vi "measure BT OCW Measurement.vi"(8 "error in (no error)":errorcluster, 11 "SA Measurement in":refnum<class "SA Measurement.lvclass">) -> (0 "error out":errorcluster, 3 "SA Measurement out":refnum<class "SA Measurement.lvclass">)   [LabVIEW 2023, in "Spectrum Analyzer.lvlib" / "SA Measurement.lvclass"]
uses:
  SA Measurement.lvclass
  SA Measurement.lvclass/SA Measurement.ctl
  TYPE DEFINITION/Keysight 9020A/TYPE Measurement Preset.ctl
  Spectrum Analyzer.lvlib
  TYPE DEFINITION/TYPE RBW and VBW Select.ctl
  Interface_Spectrum/Interface_Spectrum.lvclass
  TYPE DEFINITION/TYPE Marker Peak Search Type.ctl
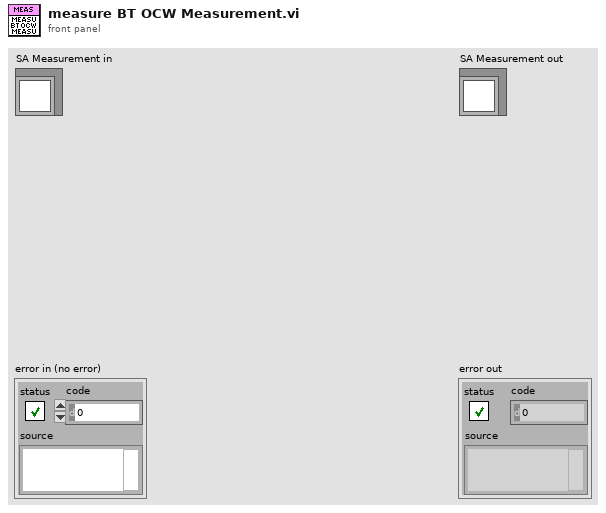
[diagram p1: front panel]
types:
  T1 = typedef "Spectrum Analyzer.lvlib/TYPE Marker Peak Search Type.ctl" = enum16{"Max", "Next Peak", "Max - Auto"}
  T2 = typedef "Spectrum Analyzer.lvlib/TYPE RBW and VBW Select.ctl" = enum16{"Res BW", "Video BW"}
  T3 = typedef "Spectrum Analyzer.lvlib/TYPE Measurement Preset.ctl" = enum16{"Sweep SA Mode", "Channel Power", "Occupied BW", "ACP", "Spurious Emission", "Spurious Emission Mask", "Burst Power (Transmit Power)"}
  T4 = typedef "Spectrum Analyzer.lvlib/TYPE Y-axis Unit.ctl" = enum16{"dBm", "dBmV", "dBuV", "dBpW", "Volt", "Ampere", "Watt"}
  T5 = typedef "Spectrum Analyzer.lvlib/TYPE Reference Level and Atten Param.ctl" = cluster{"Reference Level":dbl, "Atten":i32, "Atten Auto?":bool, "Reference Level Offset":dbl}
  T6 = typedef "Spectrum Analyzer.lvlib/TYPE Display Trace Mode Select.ctl" = enum16{"Clear Write", "Max Hold", "Min Hold", "Average", "View"}
  T7 = typedef "Spectrum Analyzer.lvlib/TYPE Detect Mode Select.ctl" = enum16{"Det Auto (Normal)", "Auto Peak", "Positive Peak", "Negative Peak", "Sample", "RMS", "Average", "Quasipeak", "CISPR Average", "RMS Average"}
  T8 = cluster{"Trace Mode":T6, "Detector Type":T7, "Detect Auto?":bool}[]
  T9 = typedef "Spectrum Analyzer.lvlib/TYPE Marker Value.ctl" = cluster{"X-axis":dbl, "Y-axis":dbl}
  T10 = typedef "Spectrum Analyzer.lvlib/TYPE OBW Measurement.ctl" = cluster{"Occupied BW (Hz)":dbl, "Total Power or OBW Power - dBm":dbl, "Transmit Frequency Error (Hz)":dbl, "x DB Bandwidth (Hz)":dbl, "Lower OBW Frequency (Hz)":dbl, "Upper OBW Frequency (Hz)":dbl}
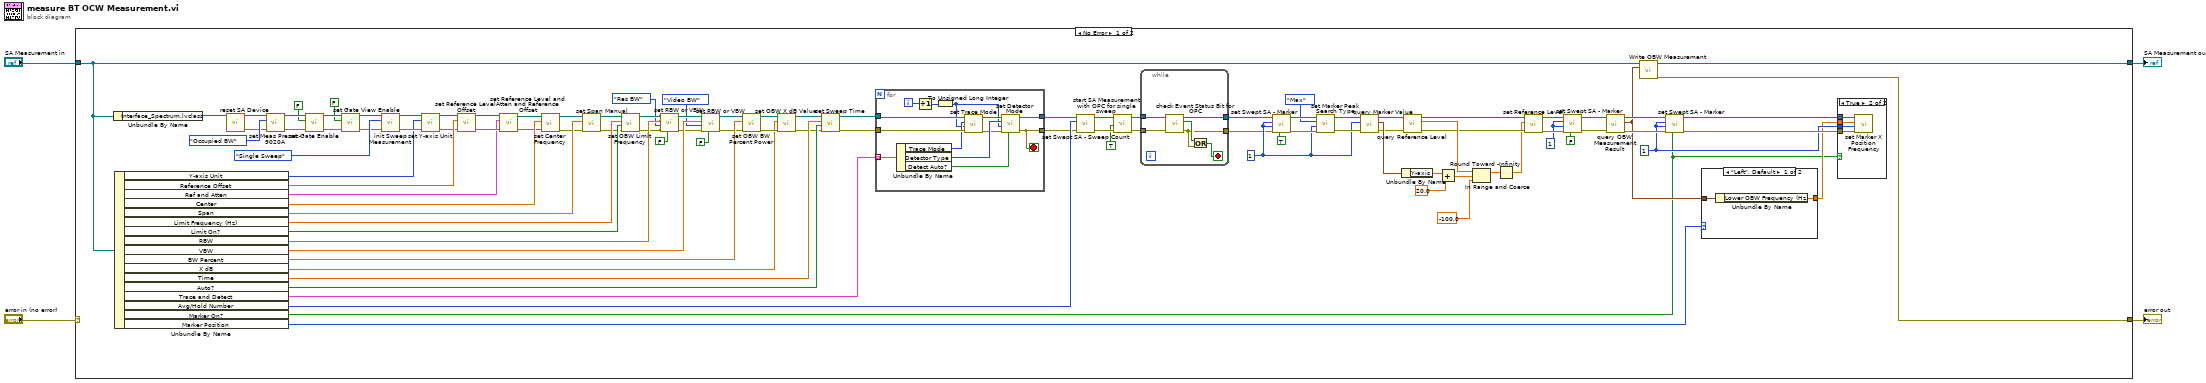
[diagram p0: block diagram]
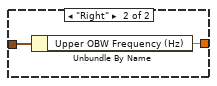
[diagram p3: hidden frame]
diagram:
  n1 = case shown="No Error" "error in (no error)" {
    selector: "error in (no error)" -> [_ w135]
    tunnel: [w58 w135] -> w3
    tunnel: [w59 w134] -> w1
    tunnel: "SA Measurement in" -> [w60 w134]
    frame No Error {
      w25 = 1 ("Index")
      w41 = 1 ("Index")
      w51 = 1 ("Index")
      n2 = Unbundle By Name(w60) -> ("Interface_Spectrum.lvclass"=w92:refnum<class "Interface_Spectrum.lvclass">)
      n3 = Unbundle By Name(w60) -> ("Y-axis Unit"=w100:T4, "Reference Offset"=w104:dbl, "Ref and Atten"=w8:T5, "Center"=w103:dbl, "Span"=w82:dbl, "Limit Frequency (Hz)"=w89:dbl, "Limit On?"=w88:bool, "RBW"=w77:dbl, "VBW"=w71:dbl, "BW Percent"=w87:dbl, "X dB"=w84:dbl, "Time"=w65:dbl, "Auto?"=w64:bool, "Trace and Detect"=w99:T8, "Avg/Hold Number"=w98:u32, "Marker On?"=w5:bool, "Marker Position"=w55:enum16{"Left", "Right"})
      n4 = call-dynamic "reset SA Device.vi"("Interface_Spectrum in"=w92) -> ("error out"=w90:errorcluster, "Interface_Spectrum out"=w91:refnum<class "Interface_Spectrum.lvclass">)  [unwired: 9 in]
      n5 = call-dynamic "set Meas Preset - 9020A.vi"("error in (no error)"=w90, "Measurement Preset"=TYPE_Measurement_Preset."Occupied BW", "Interface_Spectrum in"=w91) -> ("error out"=w19:errorcluster, "Interface_Spectrum out"=w20:refnum<class "Interface_Spectrum.lvclass">)  [unwired: 7 in]
      n6 = call-dynamic "set Gate Enable.vi"("error in (no error)"=w19, "Gate Enable"=FALSE, "Interface_Spectrum in"=w20) -> ("error out"=w16:errorcluster, "Interface_Spectrum out"=w17:refnum<class "Interface_Spectrum.lvclass">)  [unwired: 7 in]
      n7 = call-dynamic "set Gate View Enable.vi"("error in (no error)"=w16, "Gate View Enable"=FALSE, "Interface_Spectrum in"=w17) -> ("error out"=w13:errorcluster, "Interface_Spectrum out"=w14:refnum<class "Interface_Spectrum.lvclass">)  [unwired: 7 in]
      n8 = call-dynamic "init Sweep Measurement.vi"("error in (no error)"=w13, "Sweep Measurement Mode"=enum16{"Single Sweep", "Continuous Sweep"}."Single Sweep", "Interface_Spectrum in"=w14) -> ("error out"=w101:errorcluster, "Interface_Spectrum out"=w102:refnum<class "Interface_Spectrum.lvclass">)  [unwired: 7 in]
      n9 = call-dynamic "set Y-axis Unit.vi"("error in (no error)"=w101, "Y-axis Unit"=w100, "Interface_Spectrum in"=w102) -> ("error out"=w11:errorcluster, "Interface_Spectrum out"=w12:refnum<class "Interface_Spectrum.lvclass">)  [unwired: 7 in]
      n10 = call-dynamic "set Reference Level Offset.vi"("error in (no error)"=w11, "Reference Level Offset"=w104, "Interface_Spectrum in"=w12) -> ("error out"=w9:errorcluster, "Interface_Spectrum out"=w10:refnum<class "Interface_Spectrum.lvclass">)  [unwired: 7 in]
      n11 = call-dynamic "set Reference Level and Atten and Reference Offset.vi"("error in (no error)"=w9, "Reference Level, Atten, Reference Offset"=w8, "Interface_Spectrum in"=w10) -> ("error out"=w6:errorcluster, "Interface_Spectrum out"=w7:refnum<class "Interface_Spectrum.lvclass">)  [unwired: 7 in]
      n12 = call-dynamic "set Center Frequency.vi"("error in (no error)"=w6, "Center Frequency (Hz)"=w103, "Interface_Spectrum in"=w7) -> ("error out"=w81:errorcluster, "Interface_Spectrum out"=w83:refnum<class "Interface_Spectrum.lvclass">)  [unwired: 7 in]
      n13 = call-dynamic "set Span Manual.vi"("error in (no error)"=w81, "Span (Hz)"=w82, "Interface_Spectrum in"=w83) -> ("error out"=w79:errorcluster, "Interface_Spectrum out"=w80:refnum<class "Interface_Spectrum.lvclass">)  [unwired: 7 in]
      n14 = call-dynamic "set OBW Limit Frequency.vi"("error in (no error)"=w79, "Limit On?"=w88, "Limit Frequency (Hz)"=w89, "Interface_Spectrum in"=w80) -> ("error out"=w75:errorcluster, "Interface_Spectrum out"=w78:refnum<class "Interface_Spectrum.lvclass">)  [unwired: 6 in]
      n15 = call-dynamic "set RBW or VBW.vi"("BW Auto?"=FALSE, "error in (no error)"=w75, "BW Type"=TYPE_RBW_and_VBW_Select."Res BW", "BW Value (Hz)"=w77, "Interface_Spectrum in"=w78) -> ("error out"=w69:errorcluster, "Interface_Spectrum out"=w72:refnum<class "Interface_Spectrum.lvclass">)  [unwired: 5 in]
      n16 = call-dynamic "set RBW or VBW.vi"("BW Auto?"=FALSE, "error in (no error)"=w69, "BW Type"=TYPE_RBW_and_VBW_Select."Video BW", "BW Value (Hz)"=w71, "Interface_Spectrum in"=w72) -> ("error out"=w67:errorcluster, "Interface_Spectrum out"=w68:refnum<class "Interface_Spectrum.lvclass">)  [unwired: 5 in]
      n17 = call-dynamic "set OBW BW Percent Power.vi"("error in (no error)"=w67, "OBW BW % Pwr"=w87, "Interface_Spectrum in"=w68) -> ("error out"=w85:errorcluster, "Interface_Spectrum out"=w86:refnum<class "Interface_Spectrum.lvclass">)  [unwired: 7 in]
      n18 = call-dynamic "set OBW X dB Value.vi"("error in (no error)"=w85, "OBW X dB (minus Value)"=w84, "Interface_Spectrum in"=w86) -> ("error out"=w63:errorcluster, "Interface_Spectrum out"=w66:refnum<class "Interface_Spectrum.lvclass">)  [unwired: 7 in]
      n19 = call-dynamic "set Sweep Time.vi"("error in (no error)"=w63, "Sweep Time Auto?"=w64, "Sweep Time(sec)"=w65, "Interface_Spectrum in"=w66) -> ("error out"=w61:errorcluster, "Interface_Spectrum out"=w62:refnum<class "Interface_Spectrum.lvclass">)  [unwired: 6 in]
      n20 = for {
        tunnel: w62 -> [w132]
        tunnel: w61 -> [w131]
        tunnel: w99 -> [w133] mode=indexing
        tunnel: [w121] -> w48
        tunnel: [w122] -> w49
        i -> [w130]
        stop <- w121 stop-if-true
        n21 = Unbundle By Name(w133) -> ("Trace Mode"=w128:T6, "Detector Type"=w126:T7, "Detect Auto?"=w123:bool)
        n22 = Increment(x=w130) -> (x+1=w129:i32)
        n23 = To Unsigned Long Integer(number=w129) -> (unsigned 32bit integer=w124:u32)
        n24 = call-dynamic "set Trace Mode.vi"("error in (no error)"=w131, "Trace Index"=w124, "Trace Mode"=w128, "Interface_Spectrum in"=w132) -> ("error out"=w125:errorcluster, "Interface_Spectrum out"=w127:refnum<class "Interface_Spectrum.lvclass">)  [unwired: 6 in]
        n25 = call-dynamic "set Detector Mode.vi"("Detect Auto?"=w123, "error in (no error)"=w125, "Trace Index"=w124, "Detector Type"=w126, "Interface_Spectrum in"=w127) -> ("error out"=w121:errorcluster, "Interface_Spectrum out"=w122:refnum<class "Interface_Spectrum.lvclass">)  [unwired: 5 in]
      }
      n26 = call-dynamic "set Swept SA - Sweep Count.vi"("error in (no error)"=w48, "Sweep Count"=w98, "Interface_Spectrum in"=w49) -> ("error out"=w96:errorcluster, "Interface_Spectrum out"=w97:refnum<class "Interface_Spectrum.lvclass">)  [unwired: 7 in]
      n27 = call-dynamic "start SA Measurement with OPC for single sweep.vi"("error in (no error)"=w96, "with OPC?"=TRUE, "Interface_Spectrum in"=w97) -> ("error out"=w93:errorcluster, "Interface_Spectrum out"=w94:refnum<class "Interface_Spectrum.lvclass">)  [unwired: 7 in]
      n28 = while {
        tunnel: w94 -> [w120]
        tunnel: w93 -> [w119]
        tunnel: [w116] -> w23
        tunnel: [w115] -> w24
        stop <- w117 stop-if-true
        n29 = call-dynamic "check Event Status Bit for OPC.vi"("error in (no error)"=w119, "Interface_Spectrum in"=w120) -> ("error out"=w116:errorcluster, "OPC Bit Changed?"=w118:bool, "Interface_Spectrum out"=w115:refnum<class "Interface_Spectrum.lvclass">)  [unwired: 7 in]
        n30 = Or(x=w118, y=w116) -> (x .or. y?=w117:bool)
      }
      n31 = call-dynamic "set Swept SA - Marker.vi"("On?"=TRUE, "error in (no error)"=w23, "trace"=w41, "Index"=w41, "Interface_Spectrum in"=w24) -> ("error out"=w45:errorcluster, "Interface_Spectrum out"=w46:refnum<class "Interface_Spectrum.lvclass">)  [unwired: 5 in]
      n32 = call-dynamic "set Marker Peak Search Type.vi"("error in (no error)"=w45, "Marker Index"=w41, "Peak Search Type"=TYPE_Marker_Peak_Search_Type."Max", "Interface_Spectrum in"=w46) -> ("error out"=w42:errorcluster, "Interface_Spectrum out"=w43:refnum<class "Interface_Spectrum.lvclass">)  [unwired: 6 in]
      n33 = call-dynamic "query Marker Value.vi"("error in (no error)"=w42, "Marker Index"=w41, "Interface_Spectrum in"=w43) -> ("error out"=w36:errorcluster, "Marker Value"=w38:T9, "Interface_Spectrum out"=w37:refnum<class "Interface_Spectrum.lvclass">)  [unwired: 6 in]
      n34 = Unbundle By Name(w38) -> ("Y-axis"=w40:dbl)
      n35 = call-dynamic "query Reference Level.vi"("error in (no error)"=w36, "Interface_Spectrum in"=w37) -> ("error out"=w31:errorcluster, "Ref Level"=w34:dbl, "Interface_Spectrum out"=w35:refnum<class "Interface_Spectrum.lvclass">)  [unwired: 7 in]
      n36 = Add(x=w40, y=20.0) -> (x+y=w33:dbl)
      n37 = In Range and Coerce(upper limit=w34, x=w33, lower limit=-100.0) -> (coerced(x)=w30:dbl)  [unwired: 1 out]
      n38 = Round Toward -Infinity(1:w30) -> (0:w29:dbl)
      n39 = call-dynamic "set Reference Level.vi"("error in (no error)"=w31, "Reference Level"=w29, "Interface_Spectrum in"=w35) -> ("error out"=w27:errorcluster, "Interface_Spectrum out"=w28:refnum<class "Interface_Spectrum.lvclass">)  [unwired: 7 in]
      n40 = call-dynamic "set Swept SA - Marker.vi"("On?"=FALSE, "error in (no error)"=w27, "trace"=w25, "Index"=w25, "Interface_Spectrum in"=w28) -> ("error out"=w21:errorcluster, "Interface_Spectrum out"=w22:refnum<class "Interface_Spectrum.lvclass">)  [unwired: 5 in]
      n41 = call-dynamic "query OBW Measurement Result.vi"("error in (no error)"=w21, "Interface_Spectrum in"=w22) -> ("error out"=w56:errorcluster, "OBW Measurement"=w54:T10, "Interface_Spectrum out"=w57:refnum<class "Interface_Spectrum.lvclass">)  [unwired: 7 in]
      n42 = call "Write OBW Measurement.vi"("OBW Measurement"=w54, "SA Measurement in"=w60) -> ("error out"=w58:errorcluster, "SA Measurement out"=w59:refnum<class "SA Measurement.lvclass">)  [unwired: 8 in]
      n43 = call-dynamic "set Swept SA - Marker.vi"("On?"=w5, "error in (no error)"=w56, "trace"=w51, "Index"=w51, "Interface_Spectrum in"=w57) -> ("error out"=w52:errorcluster, "Interface_Spectrum out"=w53:refnum<class "Interface_Spectrum.lvclass">)  [unwired: 5 in]
      n44 = case shown="\"Left\", Default" w55 {
        tunnel: w54 -> [w112 w114]
        tunnel: [w111 w113] -> w50
        frame "Left", Default {
          n45 = Unbundle By Name(w112) -> ("Lower OBW Frequency (Hz)"=w111:dbl)
        }
        frame "Right" {
          n46 = Unbundle By Name(w114) -> ("Upper OBW Frequency (Hz)"=w113:dbl)
        }
      }
      n47 = case shown="True" w5 {
        tunnel: w53 -> [_ w110]
        tunnel: w52 -> [_ w109]
        tunnel: w51 -> [_ w108]
        tunnel: w50 -> [_ w107]
        frame False {
        }
        frame True {
          n48 = call-dynamic "set Marker X Position Frequency.vi"("error in (no error)"=w109, "Index"=w108, "X Position Frequency (Hz)"=w107, "Interface_Spectrum in"=w110) -> ()  [unwired: 6 in, 2 out]
        }
      }
    }
    frame Error {
    }
  }
  "error out" <- w3
  "SA Measurement out" <- w1
